vi "Close.vi"(8 "error in (no error)":errorcluster, 9 "timeout ms (5000)":i32=5000, 11 "WebSocket in":refnum<class "WebSocket.lvclass">) -> (0 "error out":errorcluster)   [LabVIEW 2013, in "WebSockets.lvlib" / "WebSocket.lvclass"]
doc: "Sends the close frame to the WebSocket endpoint and closes the socket connection."
uses:
  WebSocket.lvclass
  WebSocket.lvclass/WebSocket.ctl
  Sockets/Socket/Socket.lvclass
  Read Socket.vi
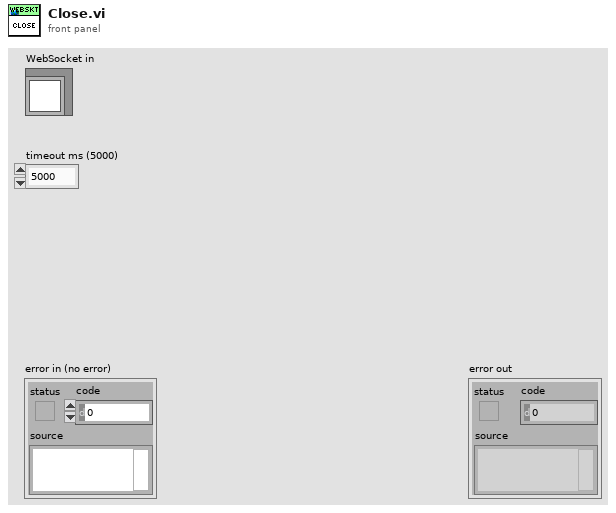
[diagram p1: front panel]
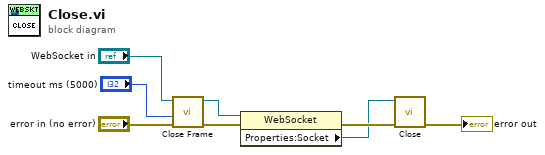
[diagram p0: block diagram]
diagram:
  n1 = call-dynamic "Close Frame.vi"("error in (no error)"="error in (no error)", "timeout ms (5000)"="timeout ms (5000)", "WebSockets in"="WebSocket in") -> ("error out"=w5:errorcluster, "WebSockets out"=w6:refnum<class "WebSocket.lvclass">)  [unwired: 7 in]
  n2 = property class="WebSocket"(reference=w6, error in=w5) -> (error out=w4:errorcluster, "Properties:Socket"=w3:refnum<class "Socket.lvclass">)  [unwired: 1 out]
  n3 = call-dynamic "Close.vi"("error in (no error)"=w4, "Socket in"=w3) -> ("error out"=→"error out":errorcluster)  [unwired: 9 in]
